vi "VIH Utility - HELP - Open Help File.vi"(6 "cmd (open)":enum16{"open", "close"}(ring), 8 "error in":errorcluster, 10 "Topic":string, 11 "Help Path":path) -> (0 "error out":errorcluster, 3 "dup Help Path":path)   [LabVIEW 2014]
doc: "::: VI Helpeks :::\nCopyright (c) 2000-2026 Konstantin Shifershteyn. All rights reserved."
panel:
  # "VI Helpeks\nCopyright (c) 2012-2026 Konstantin Shifershteyn"
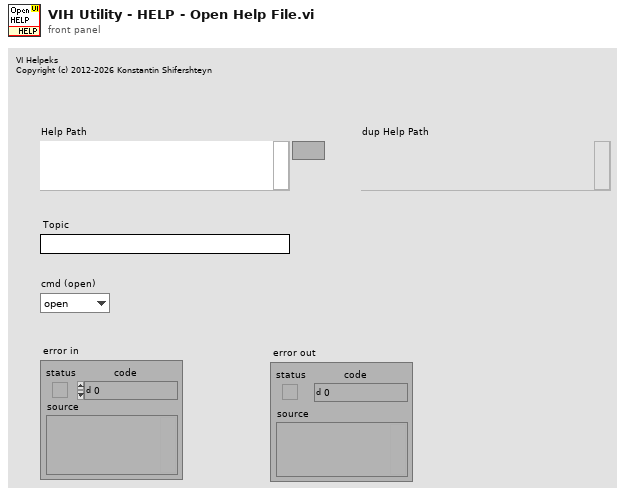
[diagram p1: front panel]
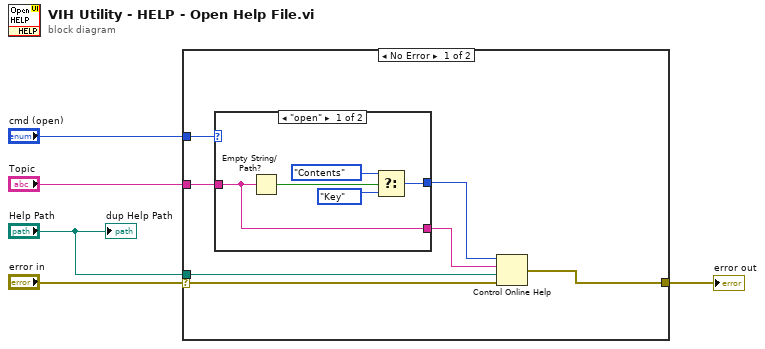
[diagram p0: block diagram]
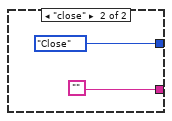
[diagram p2: hidden frame]
diagram:
  n1 = case shown="No Error" "error in" {
    selector: "error in" -> [w12 w20]
    tunnel: "Topic" -> [w9 _]
    tunnel: "Help Path" -> [w10 _]
    tunnel: [w11 w20] -> w2
    tunnel: "cmd (open)" -> [w7 _]
    frame No Error {
      n2 = case shown="\"open\"" w7 {
        tunnel: w9 -> [w13 _]
        tunnel: [w14 enum16{"Contents", "Key", "Close"}."Close" ("Operation")] -> w8
        tunnel: [w13 ""] -> w6
        frame "open" {
          n3 = Empty String/Path?(string/path=w13) -> (empty?=w16:bool)
          n4 = Select(t=enum16{"Contents", "Key", "Close"}."Contents" ("Operation"), s=w16, f=enum16{"Contents", "Key", "Close"}."Key" ("Operation")) -> (s? t:f=w14:enum16{"Contents", "Key", "Close"})
        }
        frame "close" {
        }
      }
      n5 = Control Online Help(1:w12, 2:w10, 3:w6, 4:w8) -> (0:w11:errorcluster)
    }
    frame Error {
    }
  }
  "error out" <- w2
  "dup Help Path" <- "Help Path"
